vi "DSS-Tests-flatten_water_param.vi"(8 "error in":errorcluster, 11 "array variant":variant) -> (0 "error out":errorcluster, 3 "flat":dbl[](array[numeric]))   [LabVIEW 2020, in "DSS-Tests.lvlib"]
doc: "Converts the Array variant of RDC-water-generate_perm_param_to_share into its typed array (the type constant is bound to RDC-water-param.ctl) and flattens every field of every row, in order, into one 1D DBL array."
uses:
  DSS-Tests.lvlib
  Computation/RDC-water-param.ctl
  Computation/RDC-Reflection_Data_Computation.lvlib
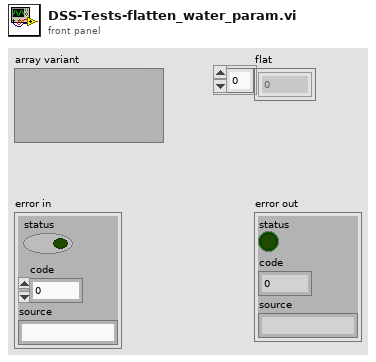
[diagram p1: front panel]
types:
  T1 = typedef "RDC-Reflection_Data_Computation.lvlib/RDC-water-param.ctl" = cluster{"temp Cx10":u16, "eps s":dbl, "eps infi":dbl, "tau":dbl, "eps s diff":dbl, "eps infi diff":dbl, "tau diff":dbl}
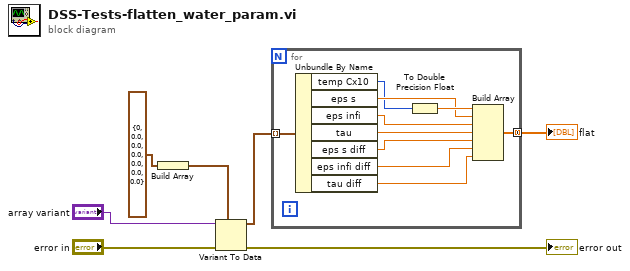
[diagram p0: block diagram]
diagram:
  n1 = Build Array(T1 {"temp Cx10"=0, "eps s"=0.0, "eps infi"=0.0, "tau"=0.0, "eps s diff"=0.0, "eps infi diff"=0.0, "tau diff"=0.0} ("water values")) -> (w4:T1[])
  n2 = Variant To Data(error in="error in", type=w4, Variant="array variant") -> (data=w5:T1[], error out=→"error out":errorcluster)
  n3 = for {
    tunnel: w5 -> [w8] mode=indexing
    tunnel: [w17] -> w7 mode=concatenating
    n4 = Unbundle By Name(w8) -> ("temp Cx10"=w9:u16, "eps s"=w10:dbl, "eps infi"=w11:dbl, "tau"=w12:dbl, "eps s diff"=w13:dbl, "eps infi diff"=w14:dbl, "tau diff"=w15:dbl)
    n5 = To Double Precision Float(number=w9) -> (double precision float=w16:dbl)
    n6 = Build Array(w16, w10, w11, w12, w13, w14, w15) -> (w17:dbl[])
  }
  "flat" <- w7
